vi "Final_output_module_ver2.vi"(0 "Toggle IN":bool=TRUE, 1 "Iteration":i32, 5 "Current Motion Output":T3, 7 "Current Motion":T2, 9 "Updated Motion Output Row":T1, 11 "Error IN":errorcluster caption="エラー定数", 12 "Instant start/stop 0 to 1":bool) -> (4 "Toggle OUT":bool, 6 "volt cluster":T5, 8 "digital cluster":T4, 10 "Feedback enabled?":bool=TRUE, 15 "Error OUT":errorcluster caption="エラー定数")   [LabVIEW 2019]
uses:
  Type_definition_current_motion.ctl
  Type_definition_updated_motion_output_row.ctl
panel:
  out "volt 1,2 2":dbl[](array[numeric])
  out "volt 3,4 2":dbl[](array[numeric])
  out "volt 5,6 2":dbl[](array[numeric])
  out "volt 1,2":dbl[](array[numeric])
  out "volt 3,4":dbl[](array[numeric])
  out "volt 5,6":dbl[](array[numeric])
  out "digital 5,6":bool[](array[boolean])
  out "digital 3,4":bool[](array[boolean])
  out "digital 1,2":bool[](array[boolean])
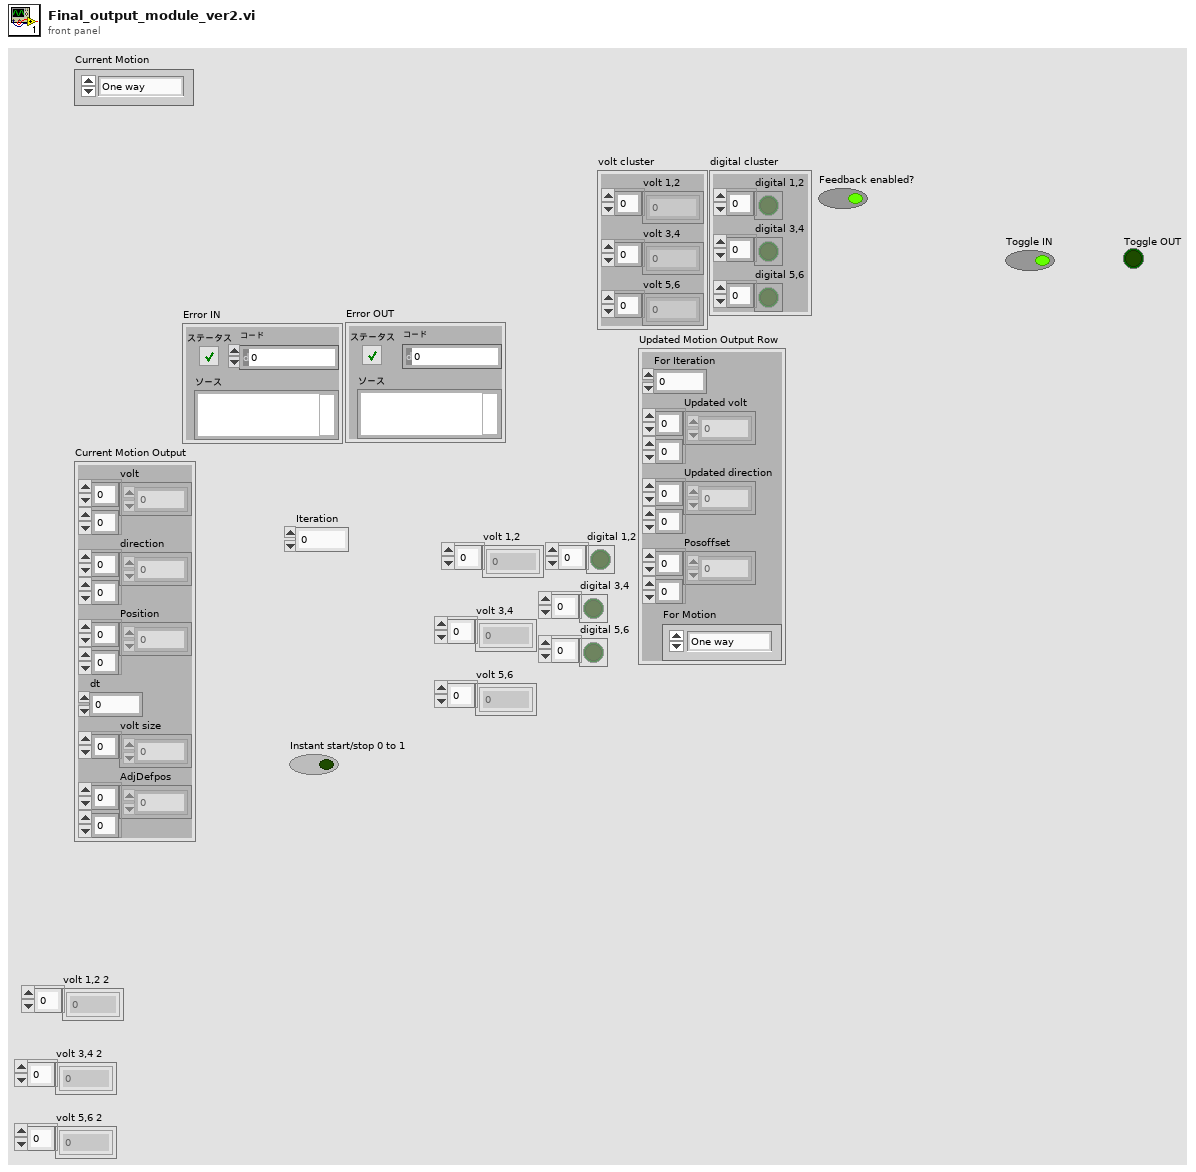
[diagram p1: front panel]
types:
  T1 = typedef "Type_definition_updated_motion_output_row.ctl" = cluster{"For Iteration":dbl, "Updated volt":dbl[][], "Updated direction":dbl[][], "Posoffset":dbl[][], "For Motion":T2}
  T2 = typedef "Type_definition_current_motion.ctl" = enum16{"One way", "Rot", "Tilt", "Tau", "XYZrot", "Zvert", "YZcirc", "Random direction tilt"}
  T3 = cluster{"volt":dbl[][], "direction":dbl[][], "Position":dbl[][], "dt":dbl, "volt size":i32[], "AdjDefpos":dbl[][]}
  T4 = cluster{"digital 1,2":bool[], "digital 3,4":bool[], "digital 5,6":bool[]}
  T5 = cluster{"volt 1,2":dbl[], "volt 3,4":dbl[], "volt 5,6":dbl[]}
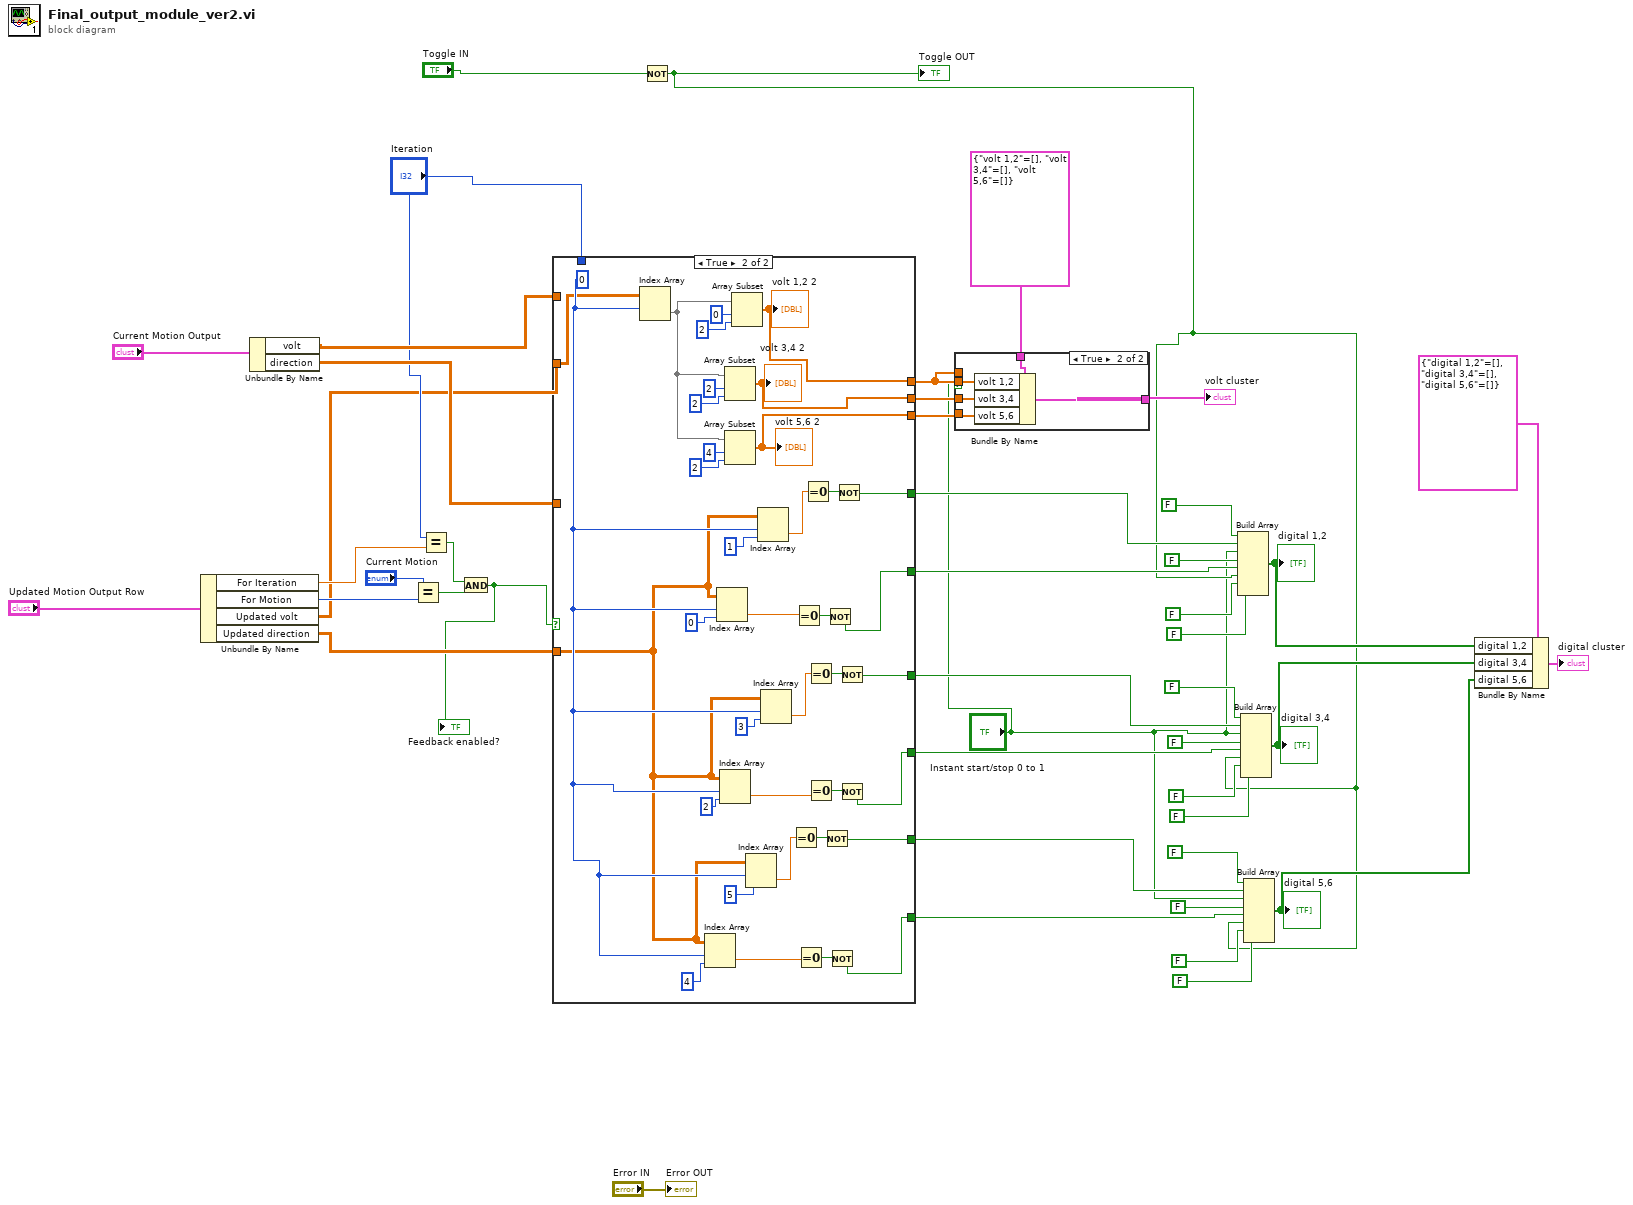
[diagram p0: block diagram]
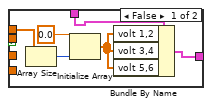
[diagram p2: hidden frame]
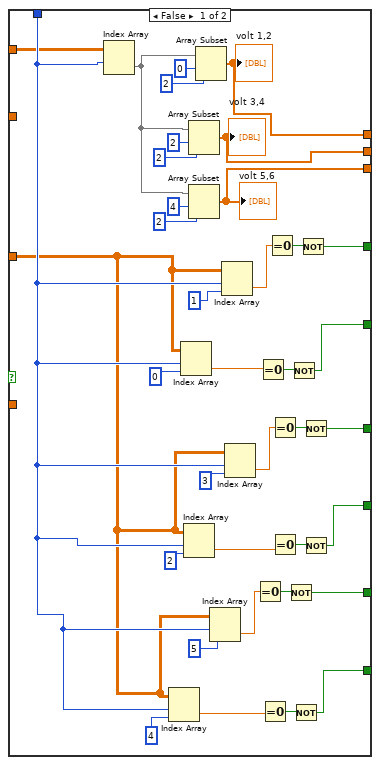
[diagram p3: hidden frame]
diagram:
  n1 = Unbundle By Name("Updated Motion Output Row") -> ("For Iteration"=w14:dbl, "For Motion"=w16:T2, "Updated volt"=w11:dbl[][], "Updated direction"=w10:dbl[][])
  n2 = Unbundle By Name("Current Motion Output") -> ("volt"=w18:dbl[][], "direction"=w17:dbl[][])
  n3 = Equal?(x="Current Motion", y=w16) -> (x = y?=w13:bool)
  n4 = Equal?(x="Iteration", y=w14) -> (x = y?=w12:bool)
  n5 = And(x=w12, y=w13) -> (x .and. y?=w6:bool)
  "Feedback enabled?" <- w6
  n6 = case shown="TRUE" w6 {
    tunnel: [w82 w86] -> w45
    tunnel: [w79 w85] -> w44
    tunnel: [w70 w89] -> w35
    tunnel: [w67 w90] -> w34
    tunnel: [w66 w88] -> w33
    tunnel: [w62 w87] -> w32
    tunnel: "Iteration" -> [w51 _]
    tunnel: [w50 w93] -> w2
    tunnel: [w49 w92] -> w26
    tunnel: [w48 w91] -> w25
    tunnel: w18 -> [w47 _]
    tunnel: w17 -> [w46 _]
    tunnel: w11 -> [_ w84]
    tunnel: w10 -> [_ w83]
    frame False {
      n7 = Index Array(array=w47, index (row)=w51) -> (element=w52:dbl[])  [unwired: 1 in]
      n8 = Index Array(array=w46, index (row)=w51, index (col)=4) -> (element=w77:dbl)
      n9 = Index Array(array=w46, index (row)=w51, index (col)=0) -> (element=w72:dbl)
      n10 = Index Array(array=w46, index (row)=w51, index (col)=2) -> (element=w60:dbl)
      n11 = Array Subset(array=w52, index=2 ("指標"), length=2 ("長さ")) -> (w49:dbl[])
      "volt 3,4" <- w49
      n12 = Array Subset(array=w52, index=4 ("指標"), length=2 ("長さ")) -> (w48:dbl[])
      "volt 5,6" <- w48
      n13 = Array Subset(array=w52, index=0 ("指標"), length=2 ("長さ")) -> (w50:dbl[])
      "volt 1,2" <- w50
      n14 = Index Array(array=w46, index (row)=w51, index (col)=5) -> (element=w81:dbl)
      n15 = Index Array(array=w46, index (row)=w51, index (col)=1) -> (element=w68:dbl)
      n16 = Index Array(array=w46, index (row)=w51, index (col)=3) -> (element=w65:dbl)
      n17 = Equal To 0?(x=w81) -> (x = 0?=w80:bool)
      n18 = Equal To 0?(x=w72) -> (x = 0?=w71:bool)
      n19 = Equal To 0?(x=w77) -> (x = 0?=w78:bool)
      n20 = Equal To 0?(x=w68) -> (x = 0?=w69:bool)
      n21 = Equal To 0?(x=w65) -> (x = 0?=w64:bool)
      n22 = Equal To 0?(x=w60) -> (x = 0?=w61:bool)
      n23 = Not(x=w80) -> (.not. x?=w82:bool)
      n24 = Not(x=w71) -> (.not. x?=w70:bool)
      n25 = Not(x=w78) -> (.not. x?=w79:bool)
      n26 = Not(x=w69) -> (.not. x?=w67:bool)
      n27 = Not(x=w64) -> (.not. x?=w66:bool)
      n28 = Not(x=w61) -> (.not. x?=w62:bool)
    }
    frame True {
      w94 = 0 ("指標 (行)")
      n29 = Index Array(array=w84, index (row)=w94) -> (element=w107:dbl[])  [unwired: 1 in]
      n30 = Index Array(array=w83, index (row)=w94, index (col)=4) -> (element=w116:dbl)
      n31 = Index Array(array=w83, index (row)=w94, index (col)=0) -> (element=w115:dbl)
      n32 = Index Array(array=w83, index (row)=w94, index (col)=2) -> (element=w108:dbl)
      n33 = Array Subset(array=w107, index=2 ("指標"), length=2 ("長さ")) -> (w92:dbl[])
      "volt 3,4 2" <- w92
      n34 = Array Subset(array=w107, index=4 ("指標"), length=2 ("長さ")) -> (w91:dbl[])
      "volt 5,6 2" <- w91
      n35 = Array Subset(array=w107, index=0 ("指標"), length=2 ("長さ")) -> (w93:dbl[])
      "volt 1,2 2" <- w93
      n36 = Index Array(array=w83, index (row)=w94, index (col)=5) -> (element=w119:dbl)
      n37 = Index Array(array=w83, index (row)=w94, index (col)=1) -> (element=w112:dbl)
      n38 = Index Array(array=w83, index (row)=w94, index (col)=3) -> (element=w111:dbl)
      n39 = Equal To 0?(x=w119) -> (x = 0?=w118:bool)
      n40 = Equal To 0?(x=w115) -> (x = 0?=w114:bool)
      n41 = Equal To 0?(x=w116) -> (x = 0?=w117:bool)
      n42 = Equal To 0?(x=w112) -> (x = 0?=w113:bool)
      n43 = Equal To 0?(x=w111) -> (x = 0?=w110:bool)
      n44 = Equal To 0?(x=w108) -> (x = 0?=w109:bool)
      n45 = Not(x=w118) -> (.not. x?=w86:bool)
      n46 = Not(x=w114) -> (.not. x?=w89:bool)
      n47 = Not(x=w117) -> (.not. x?=w85:bool)
      n48 = Not(x=w113) -> (.not. x?=w90:bool)
      n49 = Not(x=w110) -> (.not. x?=w88:bool)
      n50 = Not(x=w109) -> (.not. x?=w87:bool)
    }
  }
  n51 = Not(x="Toggle IN") -> (.not. x?=w8:bool)
  "Toggle OUT" <- w8
  n52 = case shown="TRUE" "Instant start/stop 0 to 1" {
    tunnel: T5 {"volt 1,2"=[], "volt 3,4"=[], "volt 5,6"=[]} -> [w120 w130]
    tunnel: w26 -> [_ w129]
    tunnel: w25 -> [_ w128]
    tunnel: [w121 w127] -> w24
    tunnel: w2 -> [_ w126]
    tunnel: w2 -> [w124 _]
    frame False {
      n53 = Array Size(array=w124) -> (size(s)=w125:i32)
      n54 = Initialize Array(0.0 ("要素"), w125) -> (w122:dbl[])
      n55 = Bundle By Name(cluster=w120, "volt 1,2"=w122, "volt 3,4"=w122, "volt 5,6"=w122) -> (w121:T5)
    }
    frame True {
      n56 = Bundle By Name(cluster=w130, "volt 1,2"=w126, "volt 3,4"=w129, "volt 5,6"=w128) -> (w127:T5)
    }
  }
  "volt cluster" <- w24
  n57 = Build Array(FALSE, w34, "Instant start/stop 0 to 1", FALSE, w35, w8, FALSE, FALSE) -> (w22:bool[])
  "digital 1,2" <- w22
  n58 = Build Array(FALSE, w33, "Instant start/stop 0 to 1", FALSE, w32, w8, FALSE, FALSE) -> (w21:bool[])
  "digital 3,4" <- w21
  n59 = Build Array(FALSE, w45, "Instant start/stop 0 to 1", FALSE, w44, w8, FALSE, FALSE) -> (w20:bool[])
  "digital 5,6" <- w20
  n60 = Bundle By Name(cluster=T4 {"digital 1,2"=[], "digital 3,4"=[], "digital 5,6"=[]}, "digital 1,2"=w22, "digital 3,4"=w21, "digital 5,6"=w20) -> (→"digital cluster":T4)
  "Error OUT" <- "Error IN"
